vi "TCP Chat Window Launcher Client.vi"() -> ()   [LabVIEW 2020]
uses:
  Chat Window/Chat Window.lvclass
  C:/Program Files/National Instruments/LabVIEW 2026/vi.lib/ActorFramework/Actor/Actor.lvclass
  Chat Window/Chat Window.lvclass/Chat Window.ctl
  Protocols/TCP Strategy/TCP Stream Initiator/TCP Stream Initiator.lvclass
  C:/Data/1_Projects/network-endpoint-actors/Source/Abstract Classes/Message Stream/Message Stream.lvclass
  <vilib>/ActorFramework/Actor/Actor.lvclass
panel:
  out "error out":errorcluster
  in  "Remote Port":u16=2001
  in  "Remote Address":string="127.0.0.1"
  # "This VI launches two instances of a chat window actor.  The two chat windows launch nested endpoints, which connect via a TCP/IP message stream.\n\n1.  (Optional)  Specify the IP address for this machine, and the IP ports for the two enpoints.\n2.  Run this VI.\n3.  Stop the application by closing either chat window.\n\nAF_Debug_Trace is set to TRUE in this project, so you can follow the action with the Desktop Execution Trace Toolkit."
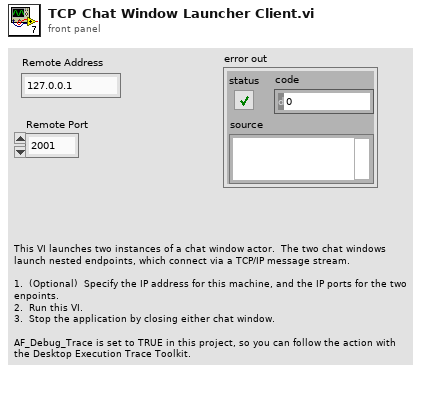
[diagram p1: front panel]
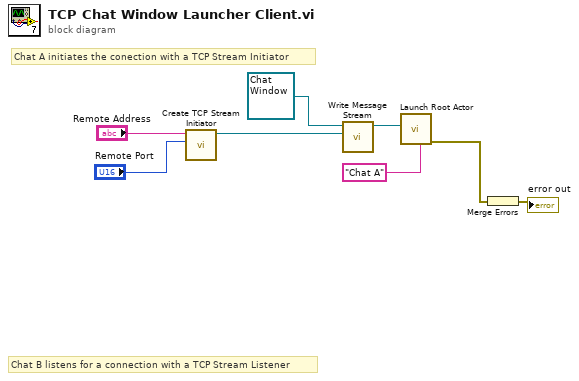
[diagram p0: block diagram]
diagram:
  # "Chat B listens for a connection with a TCP Stream Listener"
  # "Chat A initiates the conection with a TCP Stream Initiator"
  n1 = call "Create TCP Stream Initiator.vi"("Remote Port"="Remote Port", "Remote Address"="Remote Address") -> ("TCP Stream Initiator"=w6:refnum<class "TCP Stream Initiator.lvclass">)  [unwired: 9 in]
  n2 = call "Write Message Stream.vi"("Message Stream"=w6, "Chat Window in"=refnum<class "Chat Window.lvclass"> refnum) -> ("Chat Window out"=w4:refnum<class "Chat Window.lvclass">)  [unwired: 9 in]
  n3 = call <vilib>:"Launch Root Actor.vi"("Debug Alias"="Chat A", "Actor"=w4) -> ("error out"=w2:errorcluster)  [unwired: 8 in, 1 out]
  n4 = Merge Errors(w2) -> (→"error out":errorcluster)
